vi "Send Check Call Status Response.vi"(8 "error in (no error)":errorcluster caption="에러 입력(에러 없음)", 9 "connected":bool, 10 "id":string, 11 "Instrument Manager 입력":refnum<class "Instrument Manager.lvclass">) -> (0 "error out":errorcluster caption="에러 출력", 3 "Instrument Manager 출력":refnum<class "Instrument Manager.lvclass">)   [LabVIEW 2023, in "Instrument Manager.lvclass"]
uses:
  Instrument Manager.lvclass
  Check Call Status Response.ctl
  Instrument Manager.lvclass/Instrument Manager.ctl
  Error Response.ctl
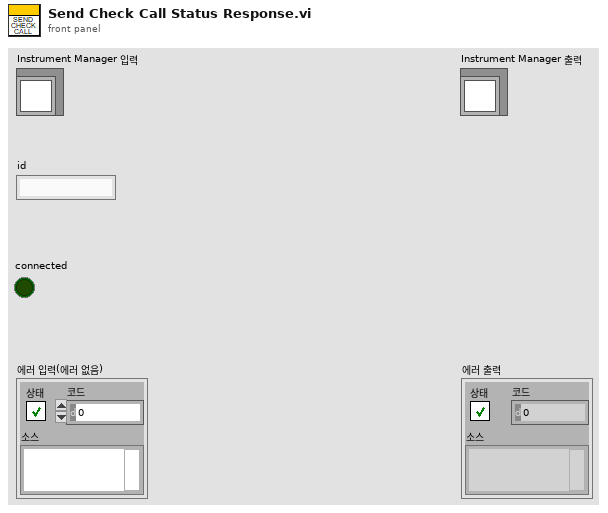
[diagram p1: front panel]
types:
  T1 = typedef "Instrument Manager.lvclass/Check Call Status Response.ctl" = cluster{"type":string, "id":string, "status":string, "Result":cluster{"ok":bool, "connected":bool}}
  T2 = cluster{"Reader Q":refnum<queue>, "Writer Q":refnum<queue>}
  T3 = typedef "Instrument Manager.lvclass/Error Response.ctl" = cluster{"type":string, "id":string, "status":string, "error out":errorcluster}
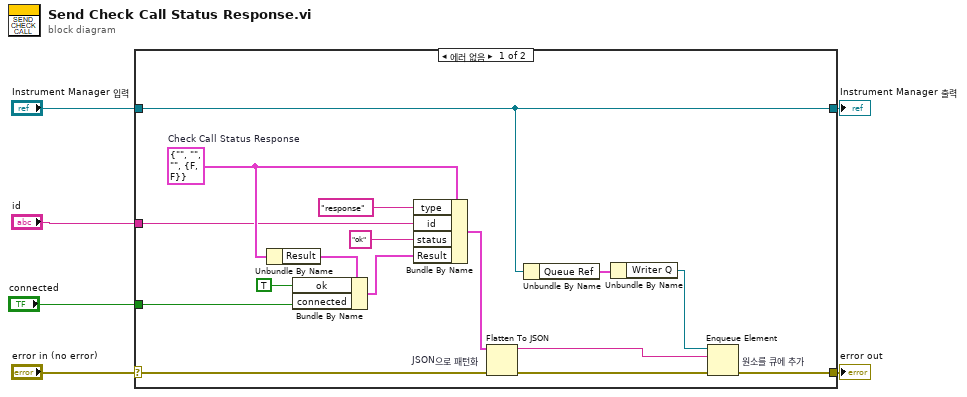
[diagram p0: block diagram]
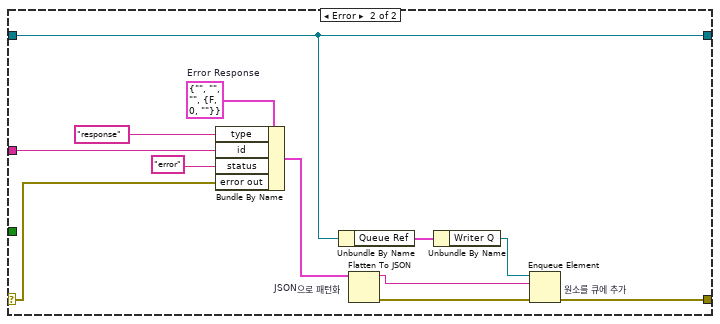
[diagram p2: hidden frame]
diagram:
  n1 = case shown="에러 없음" "error in (no error)" {
    selector: "error in (no error)" -> [w14 w32]
    tunnel: [w11 w23] -> w5
    tunnel: [w10 w24] -> w3
    tunnel: "Instrument Manager 입력" -> [w10 w24]
    tunnel: "id" -> [w18 w27]
    tunnel: "connected" -> [w17 _]
    frame No Error {
      w22 = T1 {"type"="", "id"="", "status"="", "Result"={"ok"=FALSE, "connected"=FALSE}}  # Check Call Status Response
      n2 = Unbundle By Name(w22) -> ("Result"=w21:cluster{"ok":bool, "connected":bool})
      n3 = Bundle By Name(cluster=w21, "ok"=TRUE, "connected"=w17) -> (w19:cluster{"ok":bool, "connected":bool})
      n4 = Bundle By Name(cluster=w22, "type"="response", "id"=w18, "status"="ok", "Result"=w19) -> (w13:T1)
      n5 = Flatten To JSON "JSON으로 패턴화"(anything=w13, error in (no error)=w14) -> (JSON string=w7:string, 11:w12:errorcluster)  [unwired: 1 in]
      n6 = Unbundle By Name(w10) -> ("Queue Ref"=w9:T2)
      n7 = Unbundle By Name(w9) -> ("Writer Q"=w8:refnum<queue>)
      n8 = Enqueue Element "원소를 큐에 추가"(queue=w8, element=w7, error in (no error)=w12) -> (error out=w11:errorcluster)  [unwired: 1 in, 2 out]
    }
    frame Error {
      w26 = T3 {"type"="", "id"="", "status"="", "error out"={"status"=FALSE, "code"=0, "source"=""}}  # Error Response
      n9 = Bundle By Name(cluster=w26, "type"="response", "id"=w27, "status"="error", "error out"=w32) -> (w25:T3)
      n10 = Unbundle By Name(w24) -> ("Queue Ref"=w29:T2)
      n11 = Flatten To JSON "JSON으로 패턴화"(anything=w25) -> (JSON string=w31:string, 11:w30:errorcluster)  [unwired: 2 in]
      n12 = Unbundle By Name(w29) -> ("Writer Q"=w28:refnum<queue>)
      n13 = Enqueue Element "원소를 큐에 추가"(queue=w28, element=w31, error in (no error)=w30) -> (error out=w23:errorcluster)  [unwired: 1 in, 2 out]
    }
  }
  "error out" <- w5
  "Instrument Manager 출력" <- w3
